vi "Load WAV.vi"(8 "error in (no error)":errorcluster, 11 "Path":path) -> (0 "error out":errorcluster, 1 "data":waveform(i16)[](array[waveform]), 2 "Sample Rate (Hz)":i32, 3 "Channels":i32, 5 "Length (Samples)":i32)   [LabVIEW 2019, in "Audio File Input.lvlib"]
doc: "Loads a WAV file from disk.\n\n<b>Priority:</b> Background priority (lowest)"
uses:
  Audio File Input.lvlib
  external/audio_decoder_library_wrapper/lib/audio_decoder_library_wrapper.dll
  <vilib>/sound2/lvsound2.llb/Sound File Read Open.vi
  <vilib>/sound2/lvsound2.llb/Sound File Read (I16).vi
  <vilib>/sound2/lvsound2.llb/Sound File Info (refnum).vi
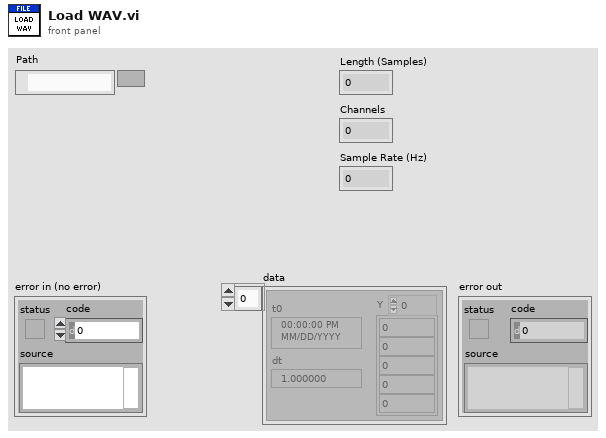
[diagram p1: front panel]
types:
  T1 = typedef "Sound File Refnum.ctl" = refnum<file>
  T2 = typedef "Sound Data Format.ctl" = cluster{"sample rate (S/s)":dbl, "number of channels":i32, "bits per sample":i32}
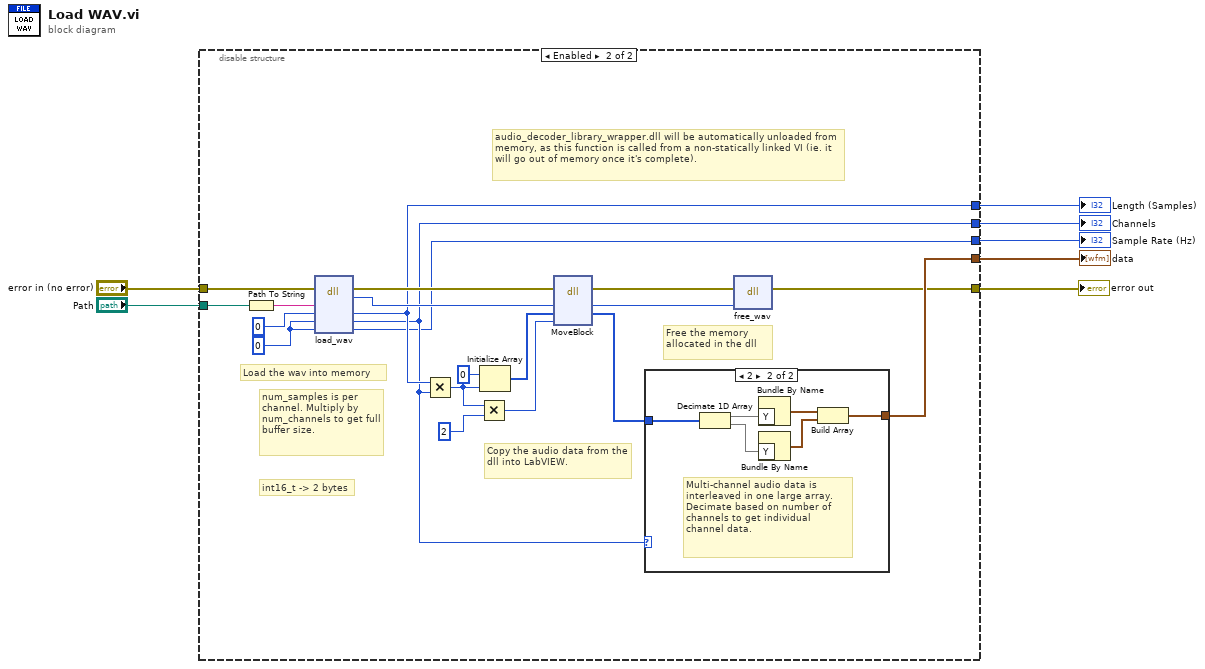
[diagram p0: block diagram]
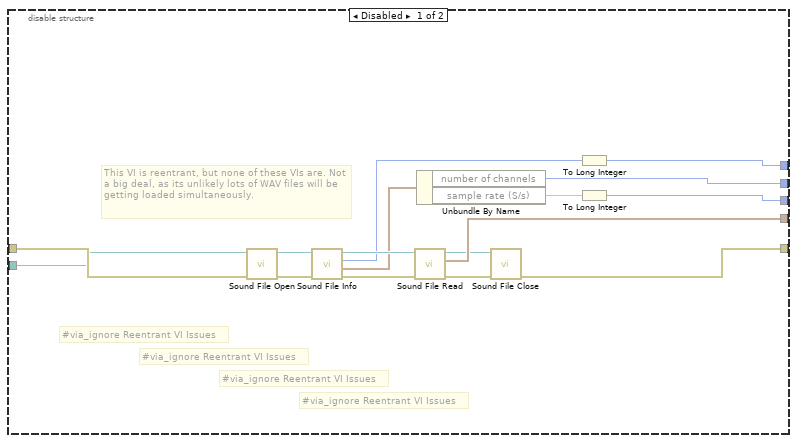
[diagram p2: hidden frame]
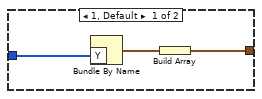
[diagram p3: hidden frame]
diagram:
  n1 = disable-structure shown="Enabled" {
    disable-tunnel: "error in (no error)" -> [w23 w29]
    disable-tunnel: [w22 w24] -> w6
    disable-tunnel: "Path" -> [w21 w30]
    disable-tunnel: [w20 w28] -> w4
    disable-tunnel: [w19 w27] -> w3
    disable-tunnel: [w18 w26] -> w2
    disable-tunnel: [w17 w25] -> w1
    frame Disabled {
      # "#via_ignore Reentrant VI Issues"
      # "#via_ignore Reentrant VI Issues"
      # "This VI is reentrant, but none of these VIs are. Not a big deal, as its unlikely lots of WAV files will be getting loaded simultaneously."
      # "#via_ignore Reentrant VI Issues"
      # "#via_ignore Reentrant VI Issues"
      n2 = call-poly <vilib>:"Sound File Open.vi"("error in (no error)"=w23, "path"=w21) -> ("error out"=w15:errorcluster, "sound file refnum"=w16:T1)  [unwired: 8 in]
      n3 = call-poly <vilib>:"Sound File Info.vi"("error in (no error)"=w15, "sound file refnum"=w16) -> ("error out"=w13:errorcluster, "sound format"=w8:T2, "total number of samples/ch"=w10:u32, "sound file refnum out"=w14:T1)  [unwired: 6 in]
      n4 = call-poly <vilib>:"Sound File Read.vi"("error in (no error)"=w13, "sound file refnum"=w14) -> ("error out"=w11:errorcluster, "data"=w17:waveform(i16)[], "sound file refnum out"=w12:T1)  [unwired: 5 in, 2 out]
      n5 = Unbundle By Name(w8) -> ("number of channels"=w19:i32, "sample rate (S/s)"=w9:dbl)
      n6 = call <vilib>:"Sound File Close.vi"("error in (no error)"=w11, "sound file refnum"=w12) -> ("error out"=w22:errorcluster)  [unwired: 9 in]
      n7 = To Long Integer(number=w10) -> (32bit integer=w20:i32)
      n8 = To Long Integer(number=w9) -> (32bit integer=w18:i32)
    }
    frame Enabled {
      w42 = u32 0 ("num_samples")
      # "audio_decoder_library_wrapper.dll will be automatically unloaded from memory, as this function is called from a non-statically linked VI (ie. it will go out of memory once it's complete)."
      # "num_samples is per channel. Multiply by num_channels to get full buffer size."
      # "Free the memory allocated in the dll"
      # "Copy the audio data from the dll into LabVIEW."
      # "Load the wav into memory"
      # "int16_t -> 2 bytes"
      n9 = Path To String(path=w30) -> (string=w43:string)
      n10 = dll-call lib="C:/github/dataflowg/dataflow-dj/external/audio_decoder_library_wrapper/lib/audio_decoder_library_wrapper.dll" fn="load_wav"(error in=w29, "file_name"=w43, "num_samples"=u64 0, "channels"=w42, "sample_rate"=w42) -> (error out=w38:errorcluster, "return type"=w40:i64, "num_samples"=w28:u64, "channels"=w27:u32, "sample_rate"=w26:u32)  [unwired: 3 in, 1 out]
      n11 = Multiply(x=w28, y=w27) -> (x*y=w31:u64)
      n12 = Multiply(x=w31, y=2) -> (x*y=w36:u64)
      n13 = Initialize Array(i16 0 ("num_samples"), w31) -> (w39:i16[])
      n14 = dll-call lib="LabVIEW" fn="MoveBlock"(error in=w38, "Address (Pointer)"=w40, "Destination"=w39, "Size"=w36) -> (error out=w34:errorcluster, "Address (Pointer)"=w35:i64, "Destination"=w33:i16[])  [unwired: 4 in, 1 out]
      n15 = case shown="2" w27 {
        tunnel: w33 -> [w46 w52]
        tunnel: [w45 w47] -> w25
        frame 1, Default {
          n16 = Bundle By Name("Y"=w46) -> (w44:waveform(i16))  [unwired: 1 in]
          n17 = Build Array(w44) -> (w45:waveform(i16)[])
        }
        frame 2 {
          # "Multi-channel audio data is interleaved in one large array. Decimate based on number of channels to get individual channel data."
          n18 = Decimate 1D Array(w52) -> (w51:i16[], w50:i16[])
          n19 = Bundle By Name("Y"=w51) -> (w49:waveform(i16))  [unwired: 1 in]
          n20 = Bundle By Name("Y"=w50) -> (w48:waveform(i16))  [unwired: 1 in]
          n21 = Build Array(w49, w48) -> (w47:waveform(i16)[])
        }
      }
      n22 = dll-call lib="C:/github/dataflowg/dataflow-dj/external/audio_decoder_library_wrapper/lib/audio_decoder_library_wrapper.dll" fn="free_wav"(error in=w34, "Address (Pointer)"=w35) -> (error out=w24:errorcluster)  [unwired: 4 in, 1 out]
    }
  }
  "error out" <- w6
  "Length (Samples)" <- w4
  "Channels" <- w3
  "Sample Rate (Hz)" <- w2
  "data" <- w1
